vi "State Delete.vi"(9 "Delete?(F)":bool, 10 "CSM name to delete":string[](array[string]), 11 "State In":string) -> (3 "State Out":string)   [LabVIEW 2026, in "UI-温度控制.lvlib"]
uses:
  <vilib>/Utility/error.llb/whitespace.ctl
  <vilib>/Utility/error.llb/Trim Whitespace (string).vi
  <vilib>/Utility/error.llb/Trim Whitespace One-Sided.vi
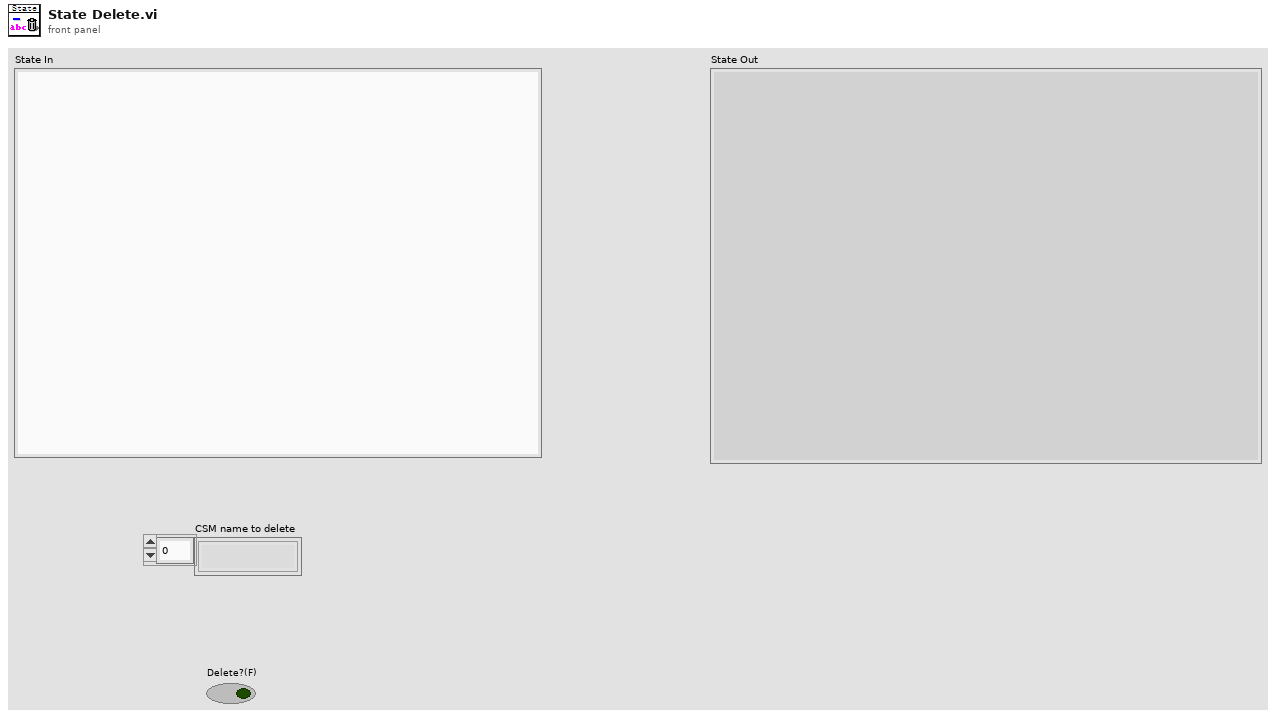
[diagram p1: front panel]
types:
  T1 = typedef "whitespace.ctl" = u16
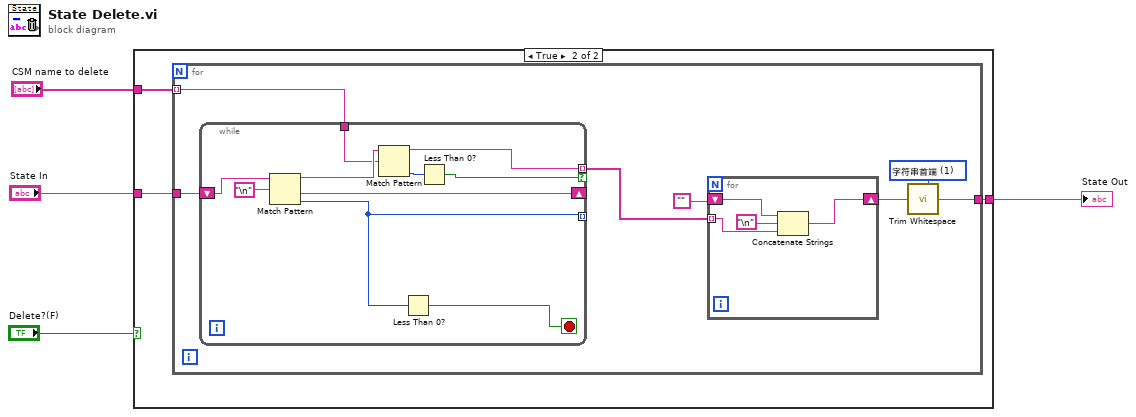
[diagram p0: block diagram]
diagram:
  n1 = case shown="True" "Delete?(F)" {
    tunnel: "State In" -> [w5 w8]
    tunnel: "CSM name to delete" -> [_ w7]
    tunnel: [w5 w6] -> w2
    frame False {
    }
    frame True {
      n2 = for {
        tunnel: w8 -> [w15]
        tunnel: w7 -> [w14] mode=indexing
        tunnel: [w13] -> w6
        w10 = T1 1 items=["两端", "字符串首端", "字符串末端"] ("location (both)")
        n3 = while {
          tunnel: [w21] -> w12 mode=indexing if=w22
          shift-right: [w27] -> _
          shift-left: w15 -> [w28]
          tunnel: w14 -> [w25]
          tunnel: [w20] -> _ mode=indexing
          stop <- w23 stop-if-true
          n4 = Match Pattern(string=w28, regular expression="\n") -> (before substring=w26:string, after substring=w27:string, offset past match=w20:i32)  [unwired: 1 in, 1 out]
          n5 = Match Pattern(string=w26, regular expression=w25) -> (before substring=w21:string, offset past match=w24:i32)  [unwired: 1 in, 2 out]
          n6 = Less Than 0?(x=w20) -> (x < 0?=w23:bool)
          n7 = Less Than 0?(x=w24) -> (x < 0?=w22:bool)
        }
        n8 = for {
          tunnel: w12 -> [w17] mode=indexing
          shift-right: [w18] -> w9
          shift-left: "" -> [w16]
          n9 = Concatenate Strings(w16, "\n", w17) -> (w18:string)
        }
        n10 = call-poly <vilib>:"Trim Whitespace.vi"("string"=w9, "location (both)"=w10) -> ("trimmed string"=w13:string)
      }
    }
  }
  "State Out" <- w2
